vi "2. Module Naming Rules.vi"() -> ()   [LabVIEW 2017]
doc: "#### Overview\n\nDemonstrates the basic string naming rules for CSM modules. A valid CSM module name is a string that should not contain any of the following special characters: `~!@%^&*()\\[\\]{}+=|\\\\/?'\"<>,.\\t\\r\\n`. These characters are keywords reserved for other purposes within the CSM framework.\n\n#### Introduction\n\nThis example demonstrates what constitutes a valid CSM module name by analyzing different scenarios.\n\n#### Steps\n\n- Step1: Regular module name.\n- Step2: Valid name containing spaces.\n- Step3: Name containing a colon (`:`).\n- Step4: Name containing a hash (`#`). In this case, the module name is valid, and the corresponding module operates in Worker Mode.\n- Step5: Name containing an underscore (`_`).\n- Step6: Name containing a hyphen (`-`).\n- Step7: Examples of invalid names containing reserved characters.\n- Step8: Name beginning with a dot (`.`). In this case, the module name is valid, and the corresponding module operates in System-Level Mode.\n- Step9: Shows a case where a dot (`.`) serves as an internal separator. In this case, the module name is valid and can be logically viewed as a Submodule.\n- Step10: Shows a case containing a dollar sign (`$`) followed by a number. In this case, the module name is valid, and the corresponding module operates in Chain Mode."
uses:
  user.lib/_NEVSTOP/Communicable State Machine(CSM)/_Support/Error/CSM Invalid Name Error.vi
  user.lib/_NEVSTOP/Communicable State Machine(CSM)/Communicable State Machine.lvlib
panel:
  in  "Module Name 11":string="module$1"
  out "error 11":errorcluster
  in  "Module Name 10":string="parent.module"
  out "error 10":errorcluster
  in  "Module Name 9":string=".module"
  out "error 9":errorcluster
  out "error 8":errorcluster={"status"=TRUE, "code"=-1, "source"="\"mod&ule\" is not a valid name."}
  in  "Module Name 8":string="mod&ule"
  out "error 7":errorcluster={"status"=TRUE, "code"=-1, "source"="\"^module\" is not a valid name."}
  out "error 6":errorcluster={"status"=TRUE, "code"=-1, "source"="\"module&name\" is not a valid name."}
  out "error 5":errorcluster
  out "error 4":errorcluster
  out "error 3":errorcluster
  out "error 2":errorcluster
  out "error 1":errorcluster
  out "error 0":errorcluster
  in  "Module Name 7":string="^module"
  in  "Module Name 6":string="module&name"
  in  "Module Name 5":string="module-name"
  in  "Module Name 4":string="module_name"
  in  "Module Name 3":string="Module#"
  in  "Module Name 2":string="Group:Module"
  in  "Module Name 1":string="module name"
  in  "Module Name 0":string="Module "
  # "#CSM-Example Overview\n\nDemonstrates the basic string naming rules for CSM modules. A valid CSM module name is a string that should not contain any of the following special characters: `~!@%^&*()\\[\\]{}+=|\\\\/?'\"<>,.\\t\\r\\n`. These characters are keywords reserved for other purposes within the CSM framework."
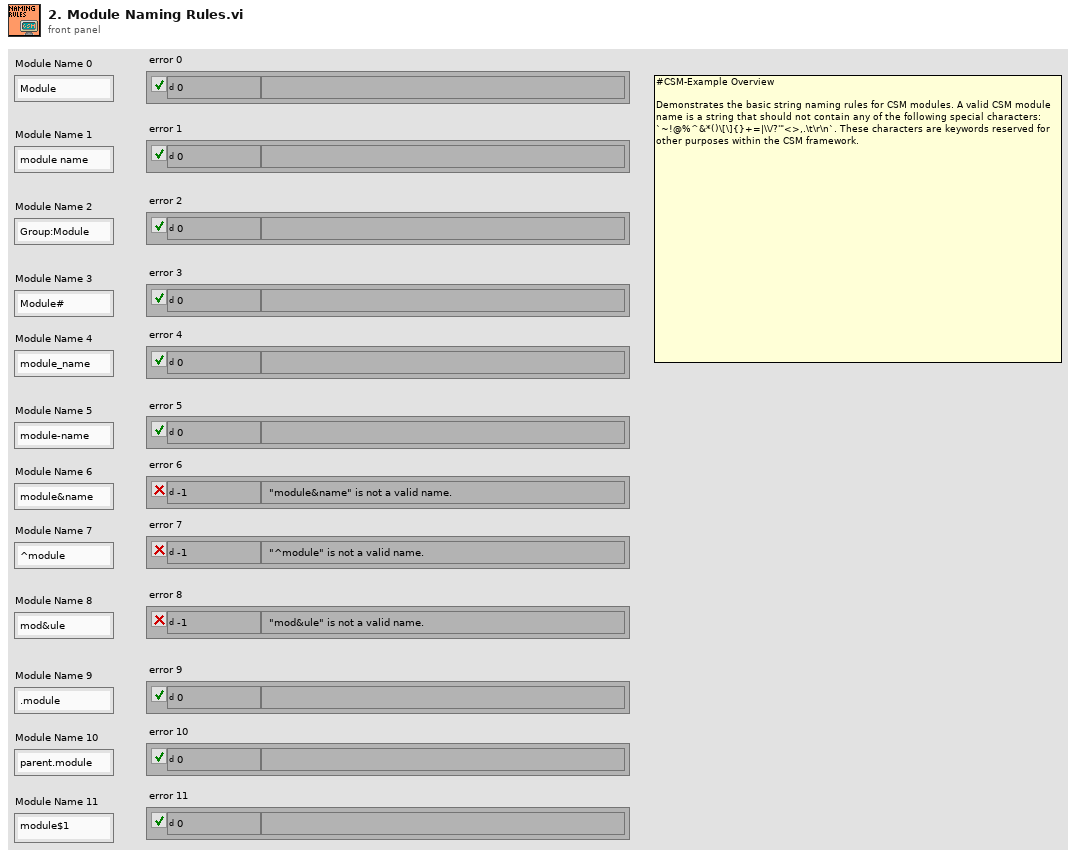
[diagram p1: front panel]
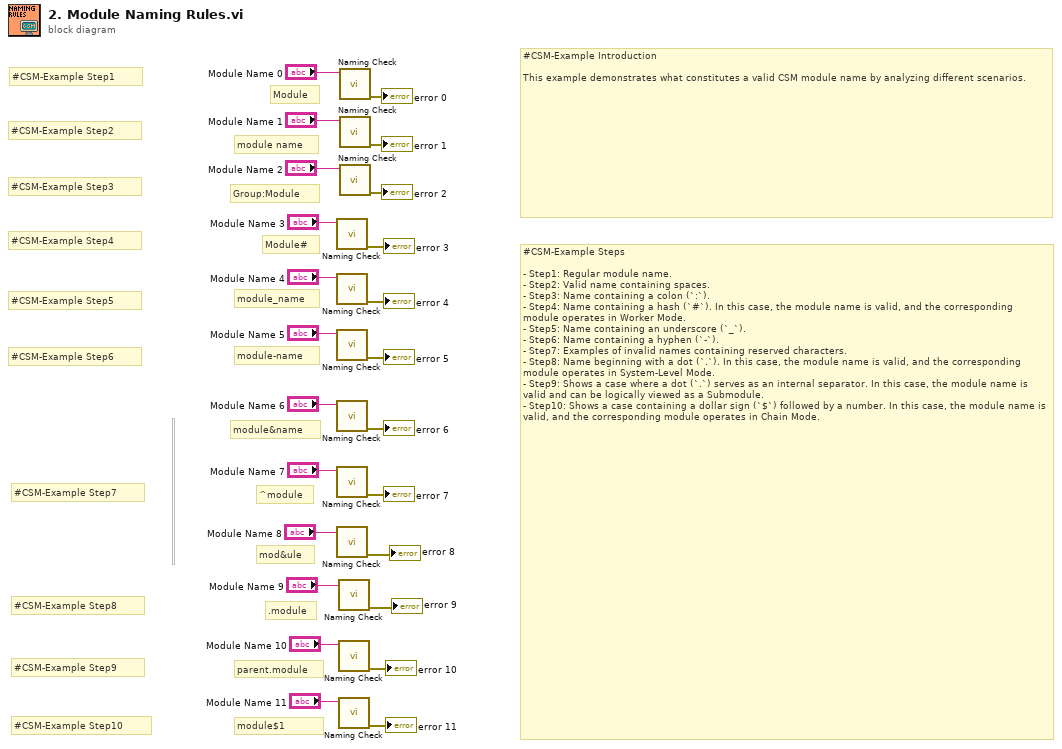
[diagram p0: block diagram]
diagram:
  # "#CSM-Example Step10"
  # "#CSM-Example Step9"
  # "#CSM-Example Step8"
  # "#CSM-Example Step7"
  # "#CSM-Example Step6"
  # "#CSM-Example Step5"
  # "#CSM-Example Step4"
  # "#CSM-Example Step3"
  # "#CSM-Example Step2"
  # "#CSM-Example Step1"
  # "module$1"
  # "parent.module"
  # ".module"
  # "mod&ule"
  # "^module"
  # "module&name"
  # "module-name"
  # "module_name"
  # "Module#"
  # "Group:Module"
  # "module name"
  # "Module"
  # "#CSM-Example Steps\n\n- Step1: Regular module name.\n- Step2: Valid name containing spaces.\n- Step3: Name containing a colon (`:`).\n- Step4: Name containing a hash (`#`). In this case, the module name is valid, and the corresponding module operates in Worker Mode.\n- Step5: Name containing an underscore (`_`).\n- Step6: Name containing a hyphen (`-`).\n- Step7: Examples of invalid names containing reserved characters.\n- Step8: Name beginning with a dot (`.`). In this case, the module name is valid, and the corresponding module operates in System-Level Mode.\n- Step9: Shows a case where a dot (`.`) serves as an internal separator. In this case, the module name is valid and can be logically viewed as a Submodule.\n- Step10: Shows a case containing a dollar sign (`$`) followed by a number. In this case, the module name is valid, and the corresponding module operates in Chain Mode."
  # "#CSM-Example Introduction\n\nThis example demonstrates what constitutes a valid CSM module name by analyzing different scenarios."
  n1 = call "Naming Check.vi"("Name (\"\" to Use UUID)"="Module Name 3") -> ("error out"=→"error 3":errorcluster)  [unwired: 9 in, 1 out]
  n2 = call "Naming Check.vi"("Name (\"\" to Use UUID)"="Module Name 4") -> ("error out"=→"error 4":errorcluster)  [unwired: 9 in, 1 out]
  n3 = call "Naming Check.vi"("Name (\"\" to Use UUID)"="Module Name 5") -> ("error out"=→"error 5":errorcluster)  [unwired: 9 in, 1 out]
  n4 = call "Naming Check.vi"("Name (\"\" to Use UUID)"="Module Name 6") -> ("error out"=→"error 6":errorcluster)  [unwired: 9 in, 1 out]
  n5 = call "Naming Check.vi"("Name (\"\" to Use UUID)"="Module Name 7") -> ("error out"=→"error 7":errorcluster)  [unwired: 9 in, 1 out]
  n6 = call "Naming Check.vi"("Name (\"\" to Use UUID)"="Module Name 8") -> ("error out"=→"error 8":errorcluster)  [unwired: 9 in, 1 out]
  n7 = call "Naming Check.vi"("Name (\"\" to Use UUID)"="Module Name 9") -> ("error out"=→"error 9":errorcluster)  [unwired: 9 in, 1 out]
  n8 = call "Naming Check.vi"("Name (\"\" to Use UUID)"="Module Name 10") -> ("error out"=→"error 10":errorcluster)  [unwired: 9 in, 1 out]
  n9 = call "Naming Check.vi"("Name (\"\" to Use UUID)"="Module Name 11") -> ("error out"=→"error 11":errorcluster)  [unwired: 9 in, 1 out]
  n10 = call "Naming Check.vi"("Name (\"\" to Use UUID)"="Module Name 0") -> ("error out"=→"error 0":errorcluster)  [unwired: 9 in, 1 out]
  n11 = call "Naming Check.vi"("Name (\"\" to Use UUID)"="Module Name 1") -> ("error out"=→"error 1":errorcluster)  [unwired: 9 in, 1 out]
  n12 = call "Naming Check.vi"("Name (\"\" to Use UUID)"="Module Name 2") -> ("error out"=→"error 2":errorcluster)  [unwired: 9 in, 1 out]
